vi "Phi Calculation(SubVI).vi"(0 "User Input Phi":dbl, 5 "Position=0, I":dbl, 7 "Up":bool, 9 "Down":bool, 11 "User Input Phi":refnum<vi>) -> (4 "Real output phi":dbl, 6 "Position=0, O":dbl, 8 "Step diff":dbl)   [LabVIEW 2018]
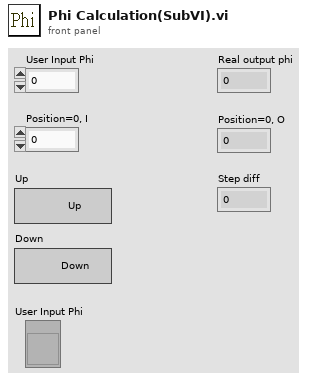
[diagram p1: front panel]
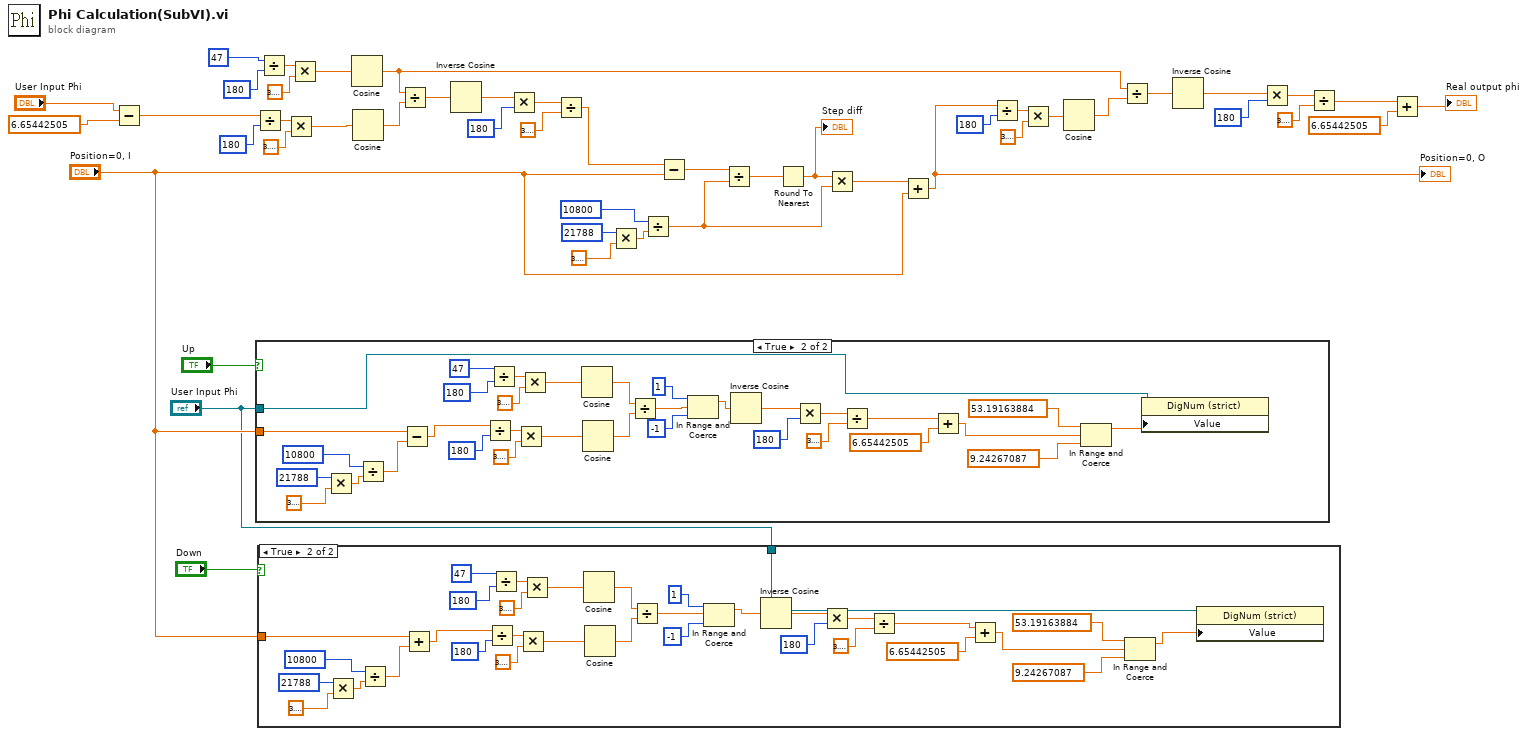
[diagram p0: block diagram]
diagram:
  n1 = Subtract(x="User Input Phi", y=6.65442505) -> (x-y=w6:dbl)
  n2 = Divide(x=w6, y=180) -> (x/y=w25:dbl)
  n3 = case shown="True" "Up" {
    tunnel: "Position=0, I" -> [_ w59]
    tunnel: "User Input Phi" -> [_ w58]
    frame False {
    }
    frame True {
      n4 = Multiply(x=21788, y=3.141592653589793) -> (x*y=w65:dbl)
      n5 = Divide(x=10800, y=w65) -> (x/y=w60:dbl)
      n6 = Subtract(x=w59, y=w60) -> (x-y=w61:dbl)
      n7 = Divide(x=w61, y=180) -> (x/y=w75:dbl)
      n8 = Divide(x=47, y=180) -> (x/y=w79:dbl)
      n9 = Multiply(x=w75, y=3.141592653589793) -> (x*y=w72:dbl)
      n10 = Multiply(x=w79, y=3.141592653589793) -> (x*y=w76:dbl)
      n11 = Cosine(x=w76) -> (cos(x)=w69:dbl)
      n12 = Cosine(x=w72) -> (cos(x)=w80:dbl)
      n13 = Divide(x=w69, y=w80) -> (x/y=w49:dbl)
      n14 = In Range and Coerce(upper limit=1, x=w49, lower limit=-1) -> (coerced(x)=w48:dbl)  [unwired: 1 out]
      n15 = Inverse Cosine(1:w48) -> (0:w71:dbl)
      n16 = Multiply(x=w71, y=180) -> (x*y=w70:dbl)
      n17 = Divide(x=w70, y=3.141592653589793) -> (x/y=w56:dbl)
      n18 = Add(x=w56, y=6.65442505) -> (x+y=w53:dbl)
      n19 = In Range and Coerce(upper limit=53.19163884, x=w53, lower limit=9.24267087) -> (coerced(x)=w52:dbl)  [unwired: 1 out]
      n20 = property class="DigNum (strict)"(reference=w58, "Value"=w52) -> ()  [unwired: 1 in, 2 out]
    }
  }
  n21 = case shown="True" "Down" {
    tunnel: "Position=0, I" -> [_ w92]
    tunnel: "User Input Phi" -> [_ w91]
    frame False {
    }
    frame True {
      n22 = Multiply(x=21788, y=3.141592653589793) -> (x*y=w98:dbl)
      n23 = Divide(x=10800, y=w98) -> (x/y=w93:dbl)
      n24 = Add(x=w92, y=w93) -> (x+y=w94:dbl)
      n25 = Divide(x=w94, y=180) -> (x/y=w108:dbl)
      n26 = Divide(x=47, y=180) -> (x/y=w112:dbl)
      n27 = Multiply(x=w108, y=3.141592653589793) -> (x*y=w105:dbl)
      n28 = Multiply(x=w112, y=3.141592653589793) -> (x*y=w109:dbl)
      n29 = Cosine(x=w109) -> (cos(x)=w102:dbl)
      n30 = Cosine(x=w105) -> (cos(x)=w113:dbl)
      n31 = Divide(x=w102, y=w113) -> (x/y=w82:dbl)
      n32 = In Range and Coerce(upper limit=1, x=w82, lower limit=-1) -> (coerced(x)=w81:dbl)  [unwired: 1 out]
      n33 = Inverse Cosine(1:w81) -> (0:w104:dbl)
      n34 = Multiply(x=w104, y=180) -> (x*y=w103:dbl)
      n35 = Divide(x=w103, y=3.141592653589793) -> (x/y=w89:dbl)
      n36 = Add(x=w89, y=6.65442505) -> (x+y=w86:dbl)
      n37 = In Range and Coerce(upper limit=53.19163884, x=w86, lower limit=9.24267087) -> (coerced(x)=w85:dbl)  [unwired: 1 out]
      n38 = property class="DigNum (strict)"(reference=w91, "Value"=w85) -> ()  [unwired: 1 in, 2 out]
    }
  }
  n39 = Divide(x=47, y=180) -> (x/y=w20:dbl)
  n40 = Multiply(x=w25, y=3.141592653589793) -> (x*y=w28:dbl)
  n41 = Multiply(x=w20, y=3.141592653589793) -> (x*y=w23:dbl)
  n42 = Cosine(x=w23) -> (cos(x)=w31:dbl)
  n43 = Cosine(x=w28) -> (cos(x)=w8:dbl)
  n44 = Divide(x=w31, y=w8) -> (x/y=w9:dbl)
  n45 = Inverse Cosine(1:w9) -> (0:w29:dbl)
  n46 = Multiply(x=w29, y=180) -> (x*y=w30:dbl)
  n47 = Divide(x=w30, y=3.141592653589793) -> (x/y=w38:dbl)
  n48 = Multiply(x=21788, y=3.141592653589793) -> (x*y=w12:dbl)
  n49 = Divide(x=10800, y=w12) -> (x/y=w16:dbl)
  n50 = Subtract(x=w38, y="Position=0, I") -> (x-y=w10:dbl)
  n51 = Divide(x=w10, y=w16) -> (x/y=w15:dbl)
  n52 = Round To Nearest(number=w15) -> (nearest integer value=w43:dbl)
  "Step diff" <- w43
  n53 = Multiply(x=w43, y=w16) -> (x*y=w17:dbl)
  n54 = Add(x=w17, y="Position=0, I") -> (x+y=w36:dbl)
  "Position=0, O" <- w36
  n55 = Divide(x=w36, y=180) -> (x/y=w32:dbl)
  n56 = Multiply(x=w32, y=3.141592653589793) -> (x*y=w35:dbl)
  n57 = Cosine(x=w35) -> (cos(x)=w18:dbl)
  n58 = Divide(x=w31, y=w18) -> (x/y=w19:dbl)
  n59 = Inverse Cosine(1:w19) -> (0:w47:dbl)
  n60 = Multiply(x=w47, y=180) -> (x*y=w37:dbl)
  n61 = Divide(x=w37, y=3.141592653589793) -> (x/y=w1:dbl)
  n62 = Add(x=w1, y=6.65442505) -> (x+y=→"Real output phi":dbl)
